vi "Test Math.vi"(8 "error in (no error)":errorcluster) -> (0 "error out":errorcluster)   [LabVIEW 2020]
doc: "This example demonstrates how to create a test suite with multiple inner test cases."
uses:
  classes/Test/Test.lvclass
  classes/Assert/Assert.lvclass
panel:
  # "See block diagram"
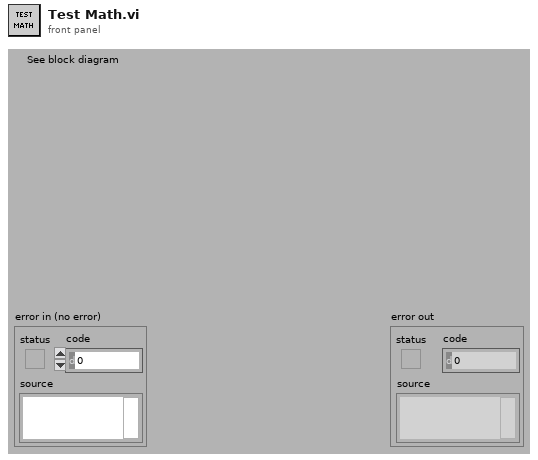
[diagram p1: front panel]
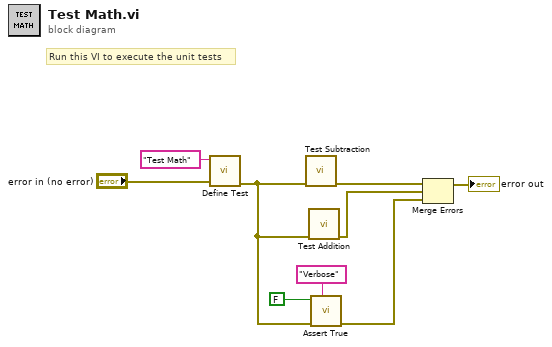
[diagram p0: block diagram]
diagram:
  # "Run this VI to execute the unit tests"
  n1 = call "Define Test.vi"("error in (no error)"="error in (no error)", "Label (VI Title)"="Test Math") -> ("error out"=w4:errorcluster)  [unwired: 8 in, 1 out]
  n2 = call "Test Subtraction.vi"("error in (no error)"=w4) -> ("error out"=w6:errorcluster)  [unwired: 10 in]
  n3 = call "Test Addition.vi"("error in (no error)"=w4) -> ("error out"=w5:errorcluster)  [unwired: 10 in]
  n4 = call "Assert True.vi"("Label"="Verbose", "error in (no error)"=w4, "True?"=FALSE) -> ("error out"=w1:errorcluster)  [unwired: 7 in, 1 out]
  n5 = Merge Errors(w6, w5, w1) -> (→"error out":errorcluster)
